vi "Create a free text label on FP.vi"(6 "Position":T1, 8 "error in (no error)":errorcluster, 10 "Text":string, 11 "Vi Reference":refnum<vi>) -> (0 "error out":errorcluster, 3 "reference out":refnum<vi>)   [LabVIEW 2012, in "Scripting Tools.lvlib"]
uses:
  Scripting Tools.lvlib
  <vilib>/Utility/miscctls.llb/LVPointTypeDef.ctl
  Private/Front Panel Object Container.vi
panel:
  # "Free Text Label"
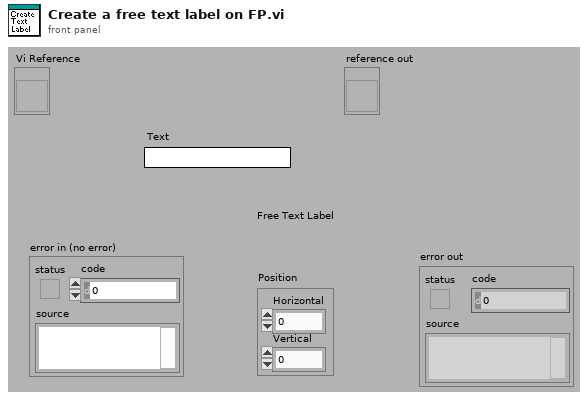
[diagram p1: front panel]
types:
  T1 = typedef "LVPointTypeDef.ctl" = cluster{"Horizontal":i16, "Vertical":i16}
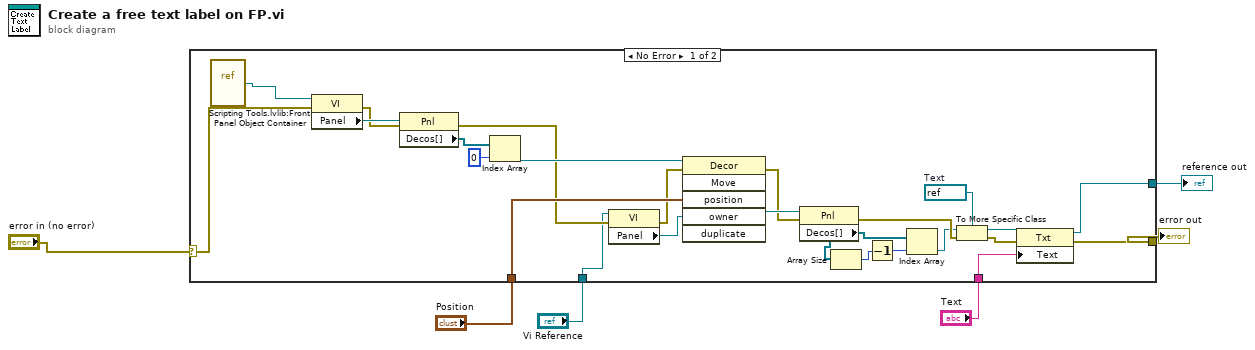
[diagram p0: block diagram]
diagram:
  n1 = case shown="No Error" "error in (no error)" {
    selector: "error in (no error)" -> [w25 w31]
    tunnel: "Position" -> [w24 _]
    tunnel: "Vi Reference" -> [w21 _]
    tunnel: "Text" -> [w10 _]
    tunnel: [w9 w31] -> w2
    tunnel: [w8 _] -> w1
    frame No Error {
      w11 = refnum<vi> refnum  # Text
      n2 = vi-ref "Scripting Tools.lvlib:Front Panel Object Container.vi"() -> (w7:refnum<vi>)
      n3 = property class="VI"(reference=w7, error in=w25) -> (error out=w29:errorcluster, "Panel"=w30:refnum<vi>)  [unwired: 1 out]
      n4 = property class="Pnl"(reference=w30, error in=w29) -> (error out=w23:errorcluster, "Decos[]"=w28:refnum<vi>[])  [unwired: 1 out]
      n5 = Index Array(array=w28, index=0) -> (element=w26:refnum<vi>)
      n6 = property class="VI"(reference=w21, error in=w23) -> (error out=w22:errorcluster, "Panel"=w20:refnum<vi>)  [unwired: 1 out]
      n7 = invoke class="Decor" method="Move"(reference=w26, error in=w22, "position"=w24, "owner"=w20) -> (error out=w19:errorcluster)  [unwired: 2 in, 5 out]
      n8 = property class="Pnl"(reference=w20, error in=w19) -> (error out=w15:errorcluster, "Decos[]"=w17:refnum<vi>[])  [unwired: 1 out]
      n9 = Array Size(array=w17) -> (size(s)=w18:i32)
      n10 = Decrement(x=w18) -> (x-1=w16:i32)
      n11 = Index Array(array=w17, index=w16) -> (element=w14:refnum<vi>)
      n12 = To More Specific Class(target class=w11, reference=w14, error in=w15) -> (specific class reference=w13:refnum<vi>, error out=w12:errorcluster)
      n13 = property class="Txt"(reference=w13, error in=w12, "Text"=w10) -> (reference out=w8:refnum<vi>, error out=w9:errorcluster)
    }
    frame Error {
    }
  }
  "error out" <- w2
  "reference out" <- w1
